vi "Center Text.vi"(8 "error in (no error)":errorcluster, 11 "Dialog in":refnum<class "Dialog.lvclass">) -> (0 "error out":errorcluster, 3 "Dialog out":refnum<class "Dialog.lvclass">)   [LabVIEW 2012, in "Dialog.lvlib" / "Dialog.lvclass"]
uses:
  Dialog.lvclass
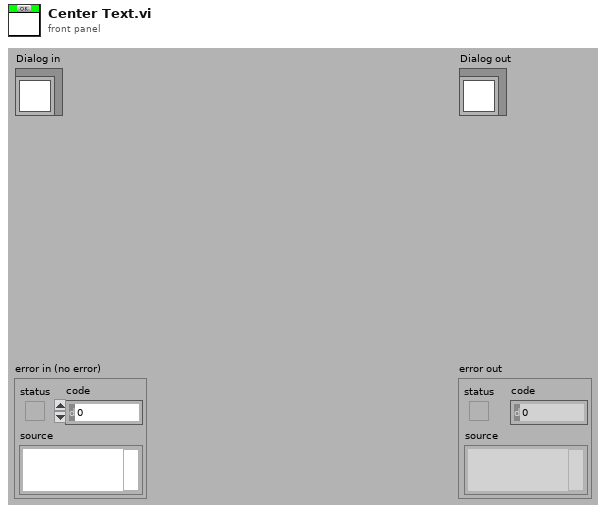
[diagram p1: front panel]
types:
  T1 = cluster{"left":i16, "top":i16, "right":i16, "bottom":i16}
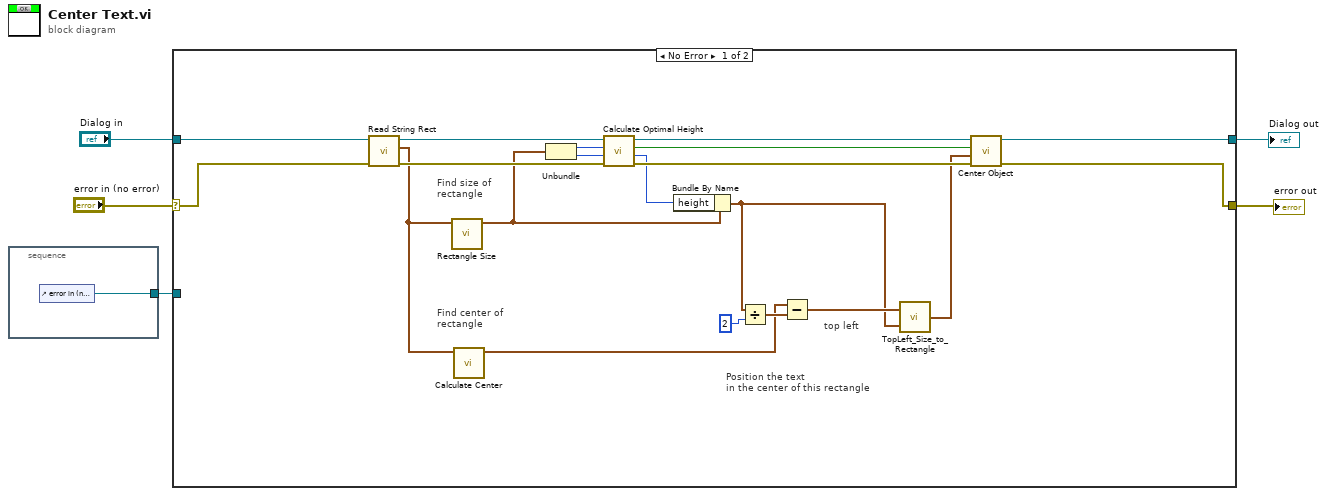
[diagram p0: block diagram]
diagram:
  n1 = stacked-sequence {
    tunnel: [w6] -> w1
    frame #0 {
      n2 = control-ref of="error in (no error)"() -> (w6:refnum<vi>)
    }
  }
  n3 = case shown="No Error" "error in (no error)" {
    selector: "error in (no error)" -> [w25 w28]
    tunnel: [w24 w28] -> w2
    tunnel: [w23 w27] -> w4
    tunnel: "Dialog in" -> [w26 w27]
    tunnel: w1 -> [_ _]
    frame No Error {
      # "top left"
      # "Find size of\nrectangle"
      # "Position the text\nin the center of this rectangle"
      # "Find center of\nrectangle"
      n4 = call-dynamic "Read String Rect.vi"("error in (no error)"=w25, "Dialog.lvclass in"=w26) -> ("error out"=w12:errorcluster, "Object Rect"=w11:T1, "Dialog.lvclass out"=w13:refnum<class "Dialog.lvclass">)  [unwired: 7 out]
      n5 = call "Rectangle Size.vi"("Rectangle"=w11) -> ("Rect Size"=w10:cluster{"width":i32, "height":i32})  [unwired: 10 out]
      n6 = call "Calculate Center.vi"("Rectangle"=w11) -> ("Center"=w21:cluster{"x":i32, "y":i32})  [unwired: 10 out]
      n7 = Unbundle(w10) -> ("width"=w15:i32, "height"=w18:i32)
      n8 = call-dynamic "Calculate Optimal Height.vi"("error in (no error)"=w12, "Max Height (200)"=w18, "Target Width (300)"=w15, "Dialog in"=w13) -> ("error out"=w16:errorcluster, "Set Height"=w14:u32, "VScrollbar Visible?"=w19:bool, "Dialog out"=w17:refnum<class "Dialog.lvclass">)  [unwired: 4 out]
      n9 = Bundle By Name(cluster=w10, "height"=w14) -> (w7:cluster{"width":i32, "height":i32})
      n10 = Divide(x=w7, y=2) -> (x/y=w22:cluster{"width":dbl, "height":dbl})
      n11 = Subtract(x=w21, y=w22) -> (x-y=w9:cluster{dbl, dbl})
      n12 = call "TopLeft_Size_to_Rectangle.vi"("Size"=w7, "Top Left"=w9) -> ("Rectangle"=w8:T1)
      n13 = call-dynamic "Center Object.vi"("error in"=w16, "Rectangle"=w8, "Scrollbar Visible?"=w19, "Dialog in"=w17) -> ("error out"=w24:errorcluster, "Dialog.lvclass out"=w23:refnum<class "Dialog.lvclass">)  [unwired: 6 out]
    }
    frame Error {
    }
  }
  "error out" <- w2
  "Dialog out" <- w4
